vi "lvmcp_gen_script_raw.vi"() -> ()   [LabVIEW 2015]
panel:
  in  "Data Strings":string[](array[string])
  in  "Type Strings":string[](array[string])
  in  "Obj Refs In[]":refnum<vi>[](array[refnum])
  out "error out":errorcluster
  out "Obj Refs Out[]":refnum<vi>[](array[refnum])
  in  "XML Script Commands":string
  in  "reference":refnum<vi>
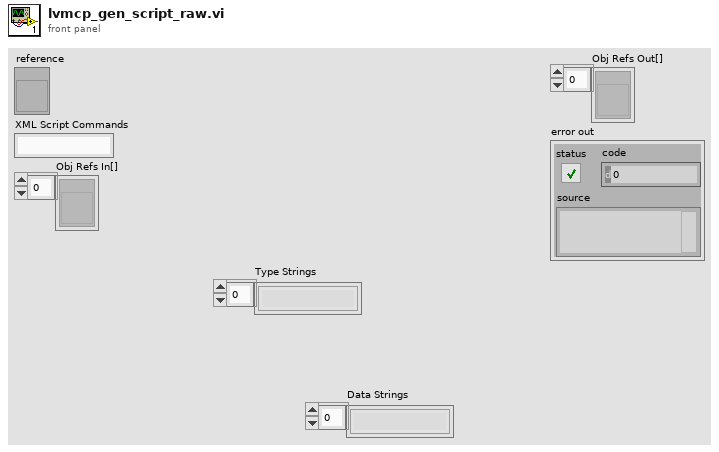
[diagram p1: front panel]
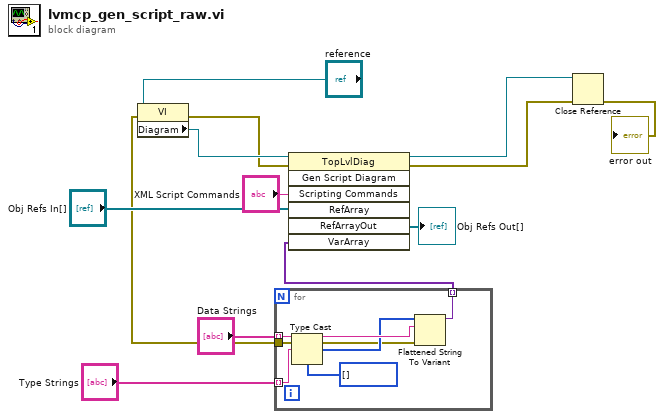
[diagram p0: block diagram]
diagram:
  n1 = for {
    tunnel: "Type Strings" -> [w18] mode=indexing
    tunnel: "Data Strings" -> [w17] mode=indexing
    tunnel: [w15] -> w4 mode=indexing
    tunnel: [w14] -> w3
    n2 = Type Cast(type=i16[] [] ("type string"), x=w18) -> (*(type *) &x=w16:i16[])
    n3 = Flattened String To Variant(6:w17, 7:w16) -> (0:w14:errorcluster, 3:w15:variant)  [unwired: 1 in]
  }
  n4 = property class="VI"(reference="reference", error in=w3) -> (error out=w11:errorcluster, "Diagram"=w12:refnum<vi>)  [unwired: 1 out]
  n5 = invoke class="TopLvlDiag" method="Gen Script Diagram"(reference=w12, error in=w11, "Scripting Commands"="XML Script Commands", "RefArray"="Obj Refs In[]", "VarArray"=w4) -> (reference out=w2:refnum<vi>, error out=w1:errorcluster, "RefArrayOut"=→"Obj Refs Out[]":refnum<vi>[])  [unwired: 2 in, 4 out]
  n6 = Close Reference(reference=w2, error in (no error)=w1) -> (error out=→"error out":errorcluster)
